vi "UE_Relative_Target_Check.vi"(8 "max_target_mm":dbl, 9 "min_target_mm":dbl, 10 "delta_mm":dbl, 11 "servo_reference_mm":dbl) -> (2 "within_limits":bool, 3 "requested_target_mm":dbl)   [LabVIEW 2026]
doc: "INTENT: Resolve relative servo motion then check authorized physical travel range. INPUTS: servo_reference_mm (double), delta_mm (double), min_target_mm (double), max_target_mm (double). OUTPUTS: requested_target_mm (double), within_limits (bool). DESIGN CONSTRAINT: Reject out-of-limit target; do not silently clamp a motion request. REQUIREMENTS: SRS-F-020, SRS-F-021. No physical hardware side effects. Acceptance requires native LabVIEW compilation and behavioral testing."
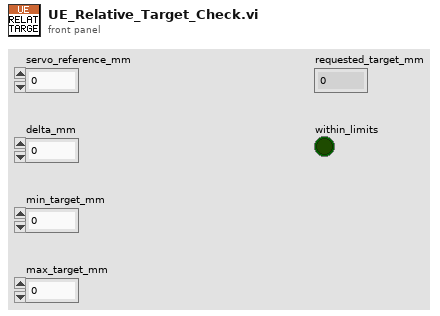
[diagram p1: front panel]
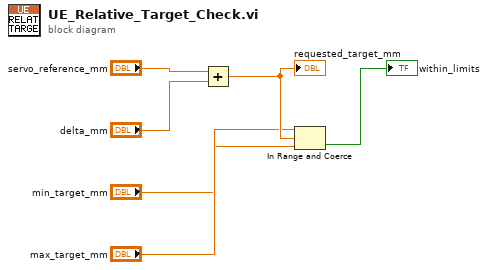
[diagram p0: block diagram]
diagram:
  n1 = Add(x="servo_reference_mm", y="delta_mm") -> (x+y=w5:dbl)
  "requested_target_mm" <- w5
  n2 = In Range and Coerce(upper limit="max_target_mm", x=w5, lower limit="min_target_mm") -> (In Range?=→"within_limits":bool)  [unwired: 1 out]
